vi "Stream Was Cancelled.vi"(8 "error in":errorcluster, 9 "request":string, 10 "cancelled":refnum<queue>, 11 "stream":string) -> (0 "error out":errorcluster, 3 "cancelled?":bool)   [LabVIEW 2020, in "MCP Server.lvlib"]
doc: "Tells Run Streamed Request.vi, after Handle MCP Request.vi has returned, whether the streamed tools/call was cancelled. cancelled? is TRUE when the cancelled flag queue of the MCP SSE Response holds TRUE (the client closed the stream or Abort Stream ran), when the state stored by Stream State.vi for this stream says so, or (legacy) when a notifications/cancelled named the id of request.\n\nWire the error out of Handle MCP Request.vi to error in: it orders the reads after the call. With an error in, the flag queue and the legacy list are not read (they count as not cancelled). error in is passed through unchanged; errors of the reads are not passed on."
uses:
  MCP Server.lvlib
  4e0c4cd1-cf2b-4ba9-b08d-62c1f8be1101.vi
  <vilib>/JDP Science/JSONtext/Next JSON Value.vi
  <vilib>/JDP Science/JSONtext/String Subset.vi
  <vilib>/JDP Science/JSONtext/Parsing/Advance past next JSON Value (inlined COPY).vi
  <vilib>/JDP Science/JSONtext/Parsing/Advance past whitespace.vi
  <vilib>/JDP Science/JSONtext/Parsing/Advance past String.vi
  <vilib>/JDP Science/JSONtext/Parsing/Advance past Number.vi
  <vilib>/JDP Science/JSONtext/Parsing/Advance past Line Ending.vi
  <vilib>/JDP Science/JSONtext/Variant to JSON Text.vi
  <vilib>/JDP Science/JSONtext/Parsing/Parse Full Path or Item Name.vi
  <vilib>/JDP Science/JSONtext/Parsing/Advance past Array.vi
  <vilib>/JDP Science/JSONtext/Parsing/Advance past Object.vi
  <vilib>/JDP Science/JSONtext/support/Error Cluster From Code.vi
  <vilib>/JDP Science/JSONtext/Offset/Find Item Locations by Path.vi
  <vilib>/JDP Science/JSONtext/LVClass Serializer/JSONtext LVClass Serializer.lvclass
  <vilib>/JDP Science/JSONtext/JSONtext.lvlib
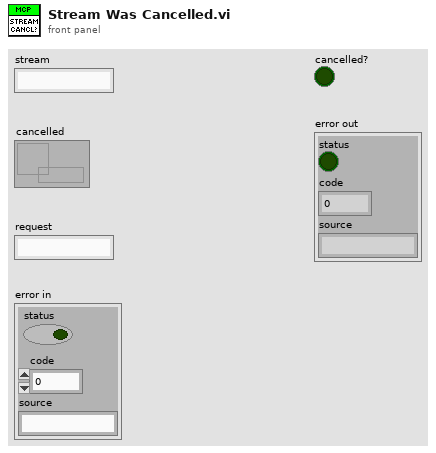
[diagram p1: front panel]
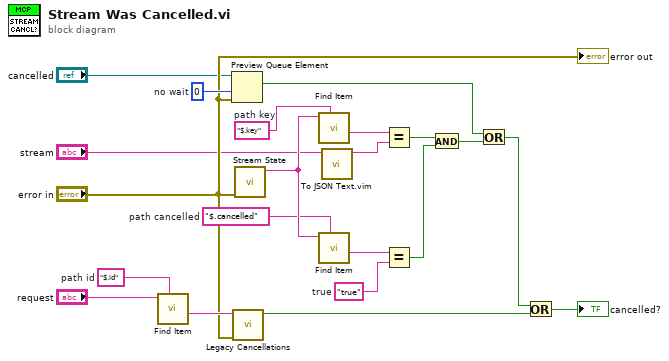
[diagram p0: block diagram]
diagram:
  w9 = "$.id"  # path id
  w8 = "true"  # true
  w7 = "$.cancelled"  # path cancelled
  w6 = "$.key"  # path key
  w5 = 0  # no wait
  n1 = call <vilib>:"Find Item.vi"("$Path or Item Name"=w9, "JSON"="request") -> ("<JSON>"=w18:string)  [unwired: 6 in, 3 out]
  n2 = Preview Queue Element(queue="cancelled", timeout in ms (-1)=w5, error in (no error)="error in") -> (element=w10:bool)  [unwired: 3 out]
  n3 = call "Legacy Cancellations.vi"("error in"="error in", "request id"=w18) -> ("recorded?"=w19:bool)  [unwired: 8 in, 1 out]
  n4 = call "Stream State.vi"("error in"="error in") -> ("state out"=w11:string)  [unwired: 9 in, 1 out]
  n5 = call <vilib>:"Find Item.vi"("$Path or Item Name"=w6, "JSON"=w11) -> ("<JSON>"=w12:string)  [unwired: 6 in, 3 out]
  n6 = call <vilib>:"Find Item.vi"("$Path or Item Name"=w7, "JSON"=w11) -> ("<JSON>"=w13:string)  [unwired: 6 in, 3 out]
  n7 = call "To JSON Text.vim"("Anything"="stream") -> ("<JSON>"=w14:string)  [unwired: 9 in, 1 out]
  n8 = Equal?(x=w12, y=w14) -> (x = y?=w15:bool)
  n9 = Equal?(x=w13, y=w8) -> (x = y?=w16:bool)
  n10 = And(x=w15, y=w16) -> (x .and. y?=w17:bool)
  n11 = Or(x=w10, y=w17) -> (x .or. y?=w20:bool)
  n12 = Or(x=w20, y=w19) -> (x .or. y?=→"cancelled?":bool)
  "error out" <- "error in"
